vi "Test U8 Change FIFO Size.vi"() -> ()   [LabVIEW 2021]
uses:
  <vilib>/CIF Foundation/CIF Channels Core/ChannelCommon/typedef/Direction.ctl
  <vilib>/CIF Foundation/CIF Channels Core/ChannelCommon/typedef/TimeStamps.ctl
  CIF_CIPC_Fifo_U8.lvclass
  D:/dev/Packages/CIF_Channels_CIPC/src/CIPC_Channels/CIF_CIPC_Chan/CIF_CIPC_Chn.lvclass
  <vilib>/CIF Foundation/CIF Channels Core/ChannelCommon/typedef/New FIFO Instance Configuration.ctl
  <vilib>/CIF Foundation/CIF Channels Core/ChannelCommon/typedef/New FIFO Config.ctl
  <vilib>/CIF Foundation/CIF Channels Core/ChannelCommon/typedef/FIFO Flags.ctl
  <vilib>/CIF Foundation/CIF Channels Core/ChannelCommon/typedef/FIFO Config.ctl
  CIF_CIPC_Chan/CIF_CIPC_Chn.lvclass
  <vilib>/CIF Foundation/CIF Channels Core/ChannelCommon/ChannelCommon.lvlib
panel:
  out "status":string
  out "pass":bool
  out "error out":errorcluster
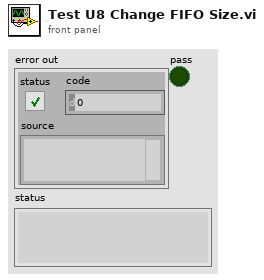
[diagram p1: front panel]
types:
  T1 = typedef "ChannelCommon.lvlib/Direction.ctl" = enum8{"Publisher", "Subscriber"}
  T2 = typedef "ChannelCommon.lvlib/New FIFO Config.ctl" = cluster{"Max Bytes/Msg":u64, "Max Msg/FIFO":u64, "FIFO Flags":T3, "Best Effort Subscribers":u32, "Backpressure Subscribers":u32}
  T3 = typedef "ChannelCommon.lvlib/FIFO Flags.ctl" = cluster{"Backpressure":bool, "Extended Config":bool}
  T4 = typedef "ChannelCommon.lvlib/New FIFO Instance Configuration.ctl" = cluster{"Backpressure":bool, "Bytes/Message Override":u32, "Messages/FIFO Override":u32, "Custom Data":u8[]}
  T5 = typedef "ChannelCommon.lvlib/TimeStamps.ctl" = cluster{"ClockID":u8, "T0":i64, "T_Out":i64}
  T6 = typedef "ChannelCommon.lvlib/FIFO Config.ctl" = cluster{"Max Bytes/Msg":u64, "Max Msg/FIFO":u64, "Flags":u64, "Custom Data":u8[]}
  T7 = typedef "ChannelCommon.lvlib/New FIFO Instance Response.ctl" = cluster{"Publisher":string, "Custom Data":u8[]}
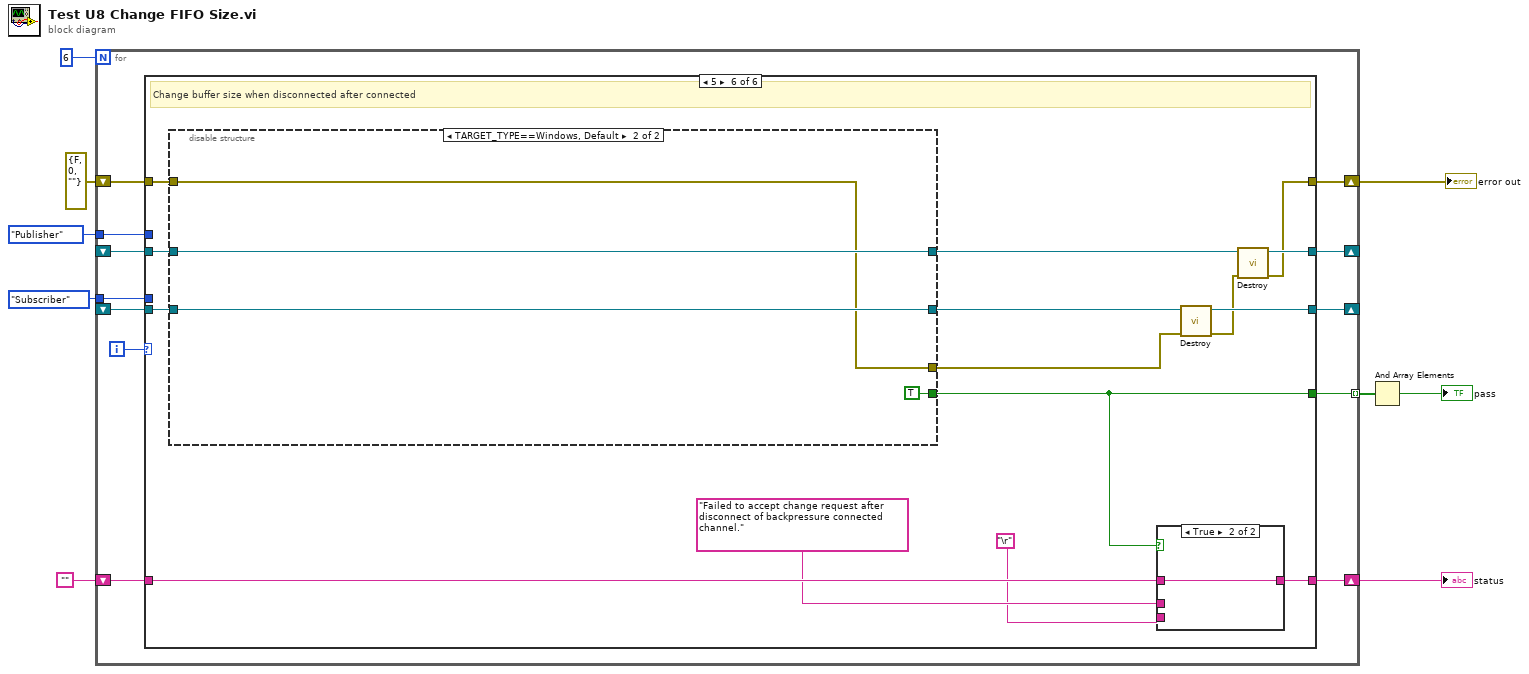
[diagram p0: block diagram]
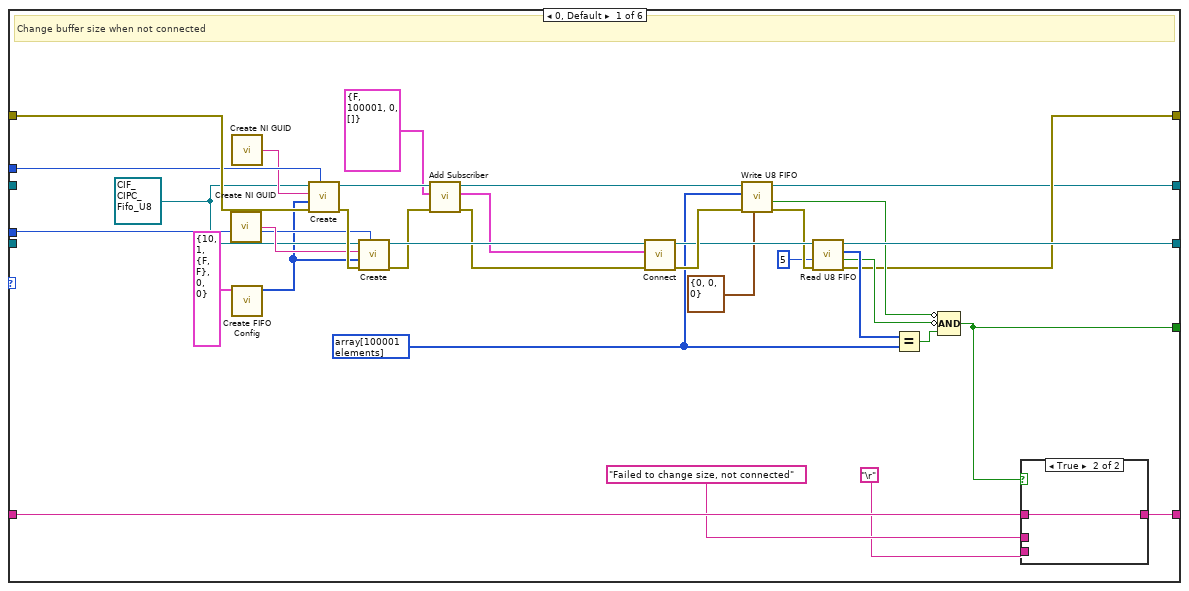
[diagram p2: hidden frame]
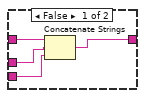
[diagram p3: hidden frame]
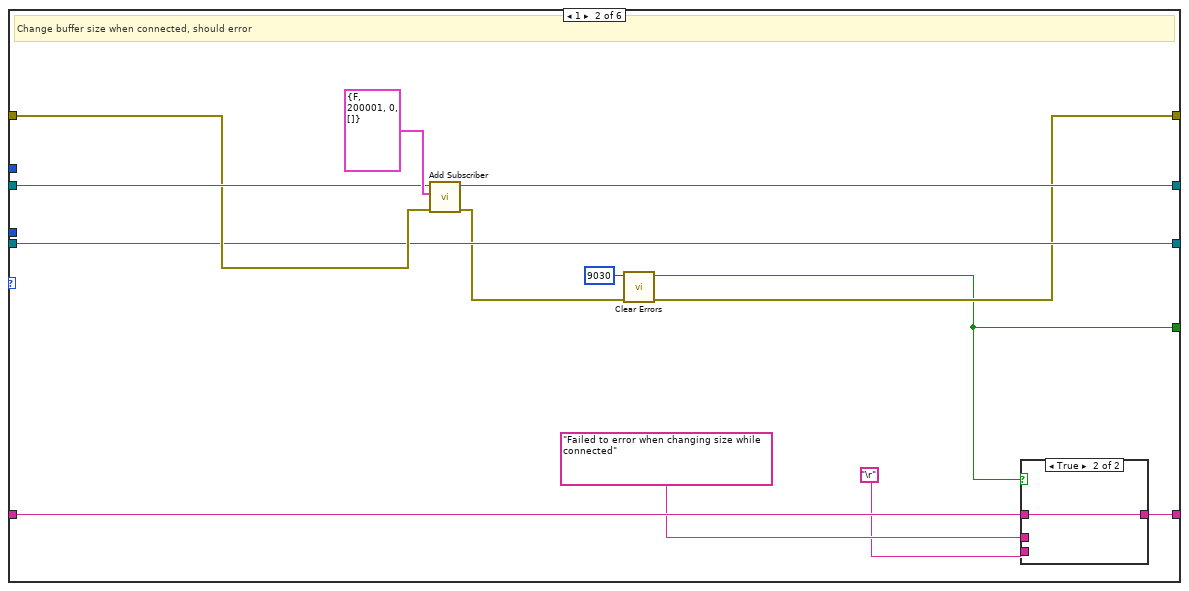
[diagram p4: hidden frame]
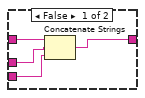
[diagram p5: hidden frame]
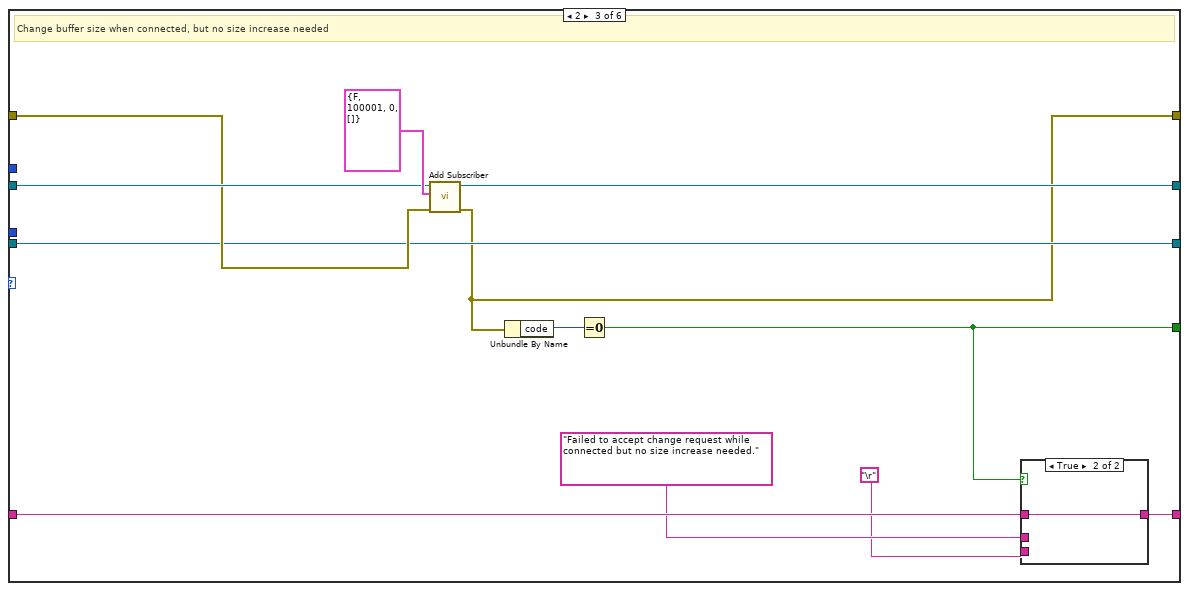
[diagram p6: hidden frame]
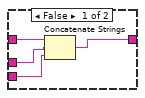
[diagram p7: hidden frame]
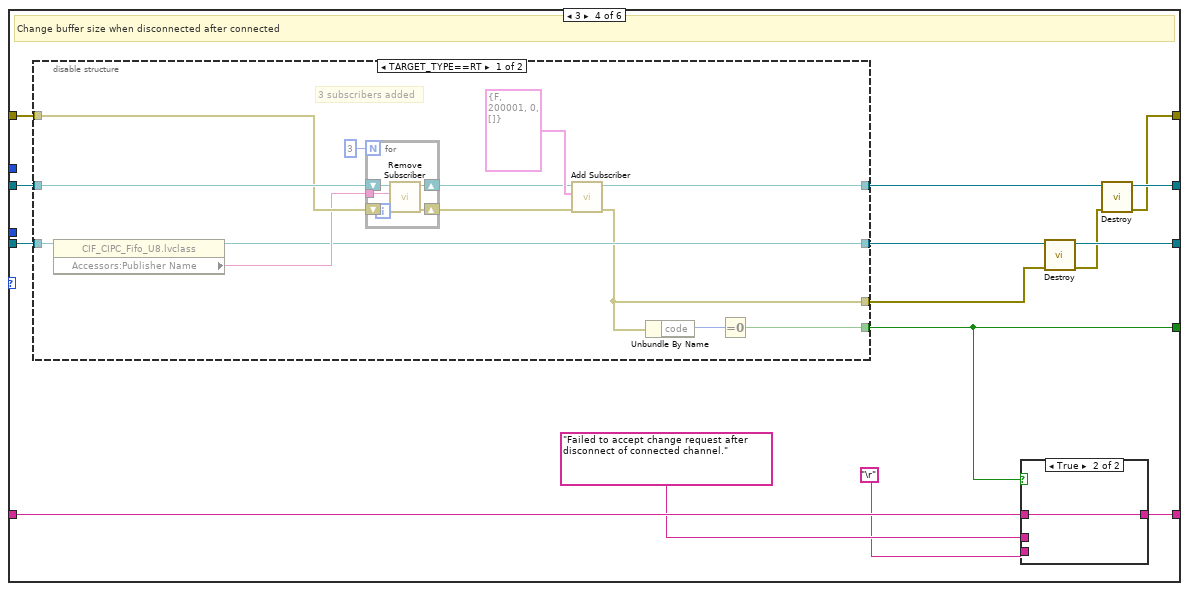
[diagram p8: hidden frame]
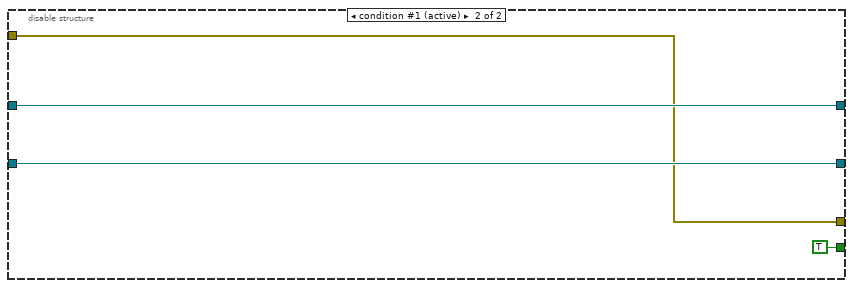
[diagram p9: hidden frame]
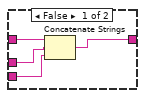
[diagram p10: hidden frame]
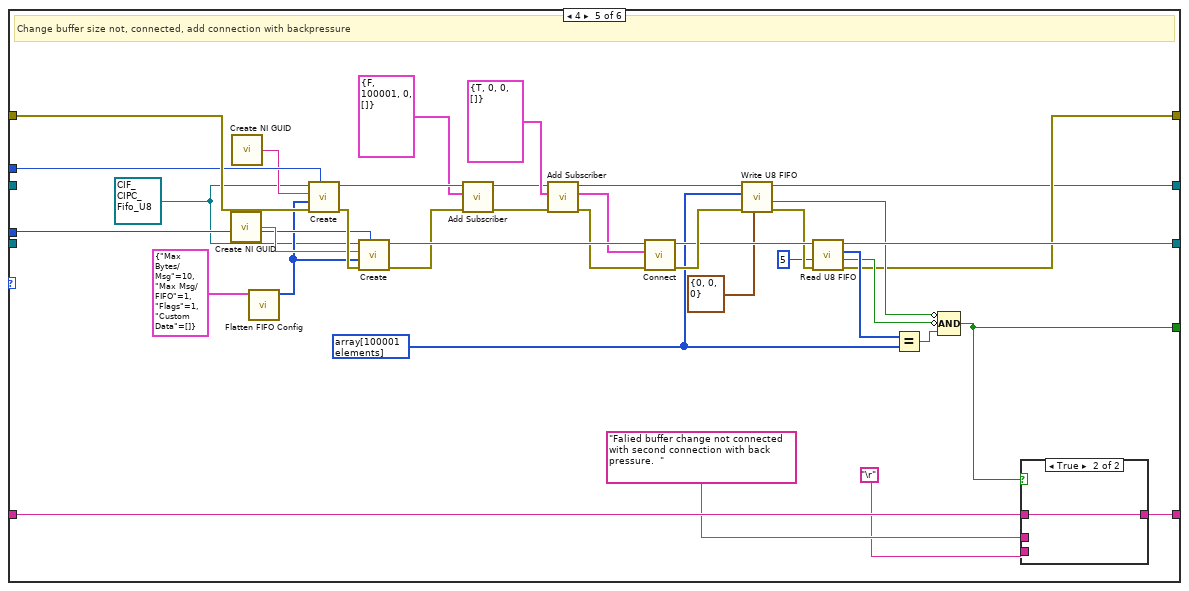
[diagram p11: hidden frame]
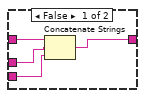
[diagram p12: hidden frame]
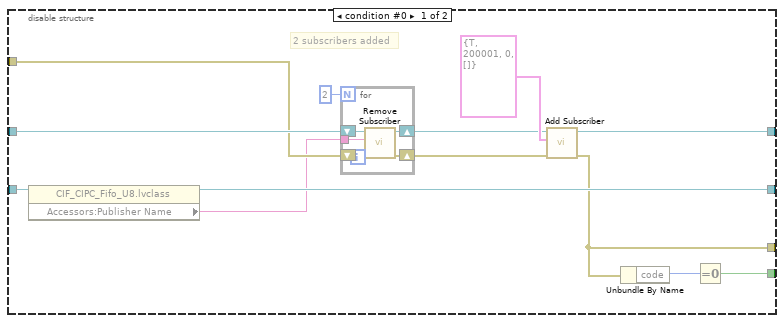
[diagram p13: hidden frame]
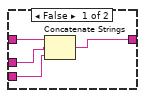
[diagram p14: hidden frame]
diagram:
  n1 = for {
    N: 6 -> [_]
    tunnel: [w21] -> w9 mode=indexing
    shift-right: [w19] -> w1
    shift-left: errorcluster {"status"=FALSE, "code"=0, "source"=""} ("error out") -> [w20]
    shift-right: [w16] -> w5
    shift-left: "" -> [w17]
    tunnel: Direction."Subscriber" ("Direction") -> [w15]
    tunnel: Direction."Publisher" ("Direction") -> [w14]
    shift-right: [w13] -> _
    shift-left: _ -> [w11]
    shift-right: [w12] -> _
    shift-left: _ -> [w10]
    i -> [w18]
    n2 = case shown="5" w18 {
      tunnel: [w50 w61 w79 w106 w169 w190] -> w21
      tunnel: w20 -> [w48 w67 w84 w104 w167 w188]
      tunnel: [w31 w63 w81 w96 w148 w180] -> w19
      tunnel: w17 -> [w55 w73 w90 w110 w174 w194]
      tunnel: [w54 w72 w89 w109 w173 w193] -> w16
      tunnel: w15 -> [w46 _ _ _ w165 _]
      tunnel: w14 -> [w45 _ _ _ w164 _]
      tunnel: [w40 w66 w83 w100 w158 w184] -> w13
      tunnel: [w30 w65 w82 w99 w147 w183] -> w12
      tunnel: w10 -> [_ w68 w85 w105 _ w189]
      tunnel: w11 -> [_ w66 w83 w103 _ w187]
      frame 0, Default {
        w35 = refnum<class "CIF_CIPC_Fifo_U8.lvclass"> refnum ("CIF_CIPC_Fifo_U8.lvclass")
        w32 = u8[] array[100001 elements] ("U8 Data")
        # "Change buffer size when not connected"
        n3 = call <vilib>:"Create NI GUID.vi"() -> ("NI GUID"=w47:string)
        n4 = call <vilib>:"Create NI GUID.vi"() -> ("NI GUID"=w44:string)
        n5 = call <vilib>:"Create FIFO Config.vi"("New FIFO Config"=T2 {"Max Bytes/Msg"=10, "Max Msg/FIFO"=1, "FIFO Flags"={"Backpressure"=FALSE, "Extended Config"=FALSE}, "Best Effort Subscribers"=0, "Backpressure Subscribers"=0}) -> ("Flattened FIFO Config"=w22:u8[])  [unwired: 10 in]
        n6 = call-dynamic "Create.vi"("Direction"=w45, "error in (no error)"=w48, "Custom Config Data"=w22, "Name"=w44, "CIFFIFO in"=w35) -> ("error out"=w49:errorcluster, "CIFFIFO out"=w29:refnum<class "CIF_CIPC_Fifo_U8.lvclass">)  [unwired: 5 in]
        n7 = call-dynamic "Create.vi"("Direction"=w46, "error in (no error)"=w49, "Custom Config Data"=w22, "Name"=w47, "CIFFIFO in"=w35) -> ("error out"=w25:errorcluster, "CIFFIFO out"=w43:refnum<class "CIF_CIPC_Fifo_U8.lvclass">)  [unwired: 5 in]
        n8 = call-dynamic "Add Subscriber.vi"("error in (no error)"=w25, "New FIFO Instance Config"=T4 {"Backpressure"=FALSE, "Bytes/Message Override"=100001, "Messages/FIFO Override"=0, "Custom Data"=[]}, "CIF_CIPC_Chn in"=w29) -> ("error out"=w24:errorcluster, "New FIFO Instance"=w27:T7, "CIF_CIPC_Chn out"=w28:refnum<class "CIF_CIPC_Fifo_U8.lvclass">)  [unwired: 6 in]
        n9 = call-dynamic "Connect.vi"("error in (no error)"=w24, "Connection"=w27, "CIFTag in"=w43) -> ("error out"=w42:errorcluster, "CIFTag out"=w41:refnum<class "CIF_CIPC_Fifo_U8.lvclass">)  [unwired: 7 in]
        n10 = call-dynamic "Write U8 FIFO.vi"("FIFO Timestamps"=T5 {"ClockID"=0, "T0"=0, "T_Out"=0}, "error in (no error)"=w42, "Data in"=w32, "CIFFIFO in"=w28) -> ("error out"=w39:errorcluster, "timed out?"=w38:bool, "CIFFIFO out"=w30:refnum<class "CIF_CIPC_Fifo_U8.lvclass">)  [unwired: 4 in, 1 out]
        n11 = call-dynamic "Read U8 FIFO.vi"("error in (no error)"=w39, "Timeout (ms)"=5, "CIFFIFO in"=w41) -> ("error out"=w31:errorcluster, "timed out?"=w36:bool, "Data out"=w37:u8[], "CIFFIFO out"=w40:refnum<class "CIF_CIPC_Fifo_U8.lvclass">)  [unwired: 4 in, 1 out]
        n12 = Equal?(x=w37, y=w32) -> (x = y?=w51:bool)
        n13 = Compound Arithmetic op=AND(invert w38, invert w36, w51) -> (w50:bool)
        n14 = case shown="True" w50 {
          tunnel: w55 -> [w59 w60]
          tunnel: [w56 w60] -> w54
          tunnel: "Failed to change size, not connected" -> [w58 _]
          tunnel: "\r" -> [w57 _]
          frame False {
            n15 = Concatenate Strings(w59, w58, w57) -> (w56:string)
          }
          frame True {
          }
        }
      }
      frame 1 {
        # "Change buffer size when connected, should error"
        n16 = call-dynamic "Add Subscriber.vi"("error in (no error)"=w67, "New FIFO Instance Config"=T4 {"Backpressure"=FALSE, "Bytes/Message Override"=200001, "Messages/FIFO Override"=0, "Custom Data"=[]}, "CIF_CIPC_Chn in"=w68) -> ("error out"=w64:errorcluster, "CIF_CIPC_Chn out"=w65:refnum<class "CIF_CIPC_Chn.lvclass">)  [unwired: 6 in, 1 out]
        n17 = call <vilib>:"Clear Errors.vi"("error in (no error)"=w64, "specific error code to clear (0: all)"=9030) -> ("error out"=w63:errorcluster, "specific error cleared?"=w61:bool)  [unwired: 4 in]
        n18 = case shown="True" w61 {
          tunnel: w73 -> [w77 w78]
          tunnel: [w74 w78] -> w72
          tunnel: "Failed to error when changing size while connected" -> [w76 _]
          tunnel: "\r" -> [w75 _]
          frame False {
            n19 = Concatenate Strings(w77, w76, w75) -> (w74:string)
          }
          frame True {
          }
        }
      }
      frame 2 {
        # "Change buffer size when connected, but no size increase needed"
        n20 = call-dynamic "Add Subscriber.vi"("error in (no error)"=w84, "New FIFO Instance Config"=T4 {"Backpressure"=FALSE, "Bytes/Message Override"=100001, "Messages/FIFO Override"=0, "Custom Data"=[]}, "CIF_CIPC_Chn in"=w85) -> ("error out"=w81:errorcluster, "CIF_CIPC_Chn out"=w82:refnum<class "CIF_CIPC_Chn.lvclass">)  [unwired: 6 in, 1 out]
        n21 = Unbundle By Name(w81) -> ("code"=w80:i32)
        n22 = Equal To 0?(x=w80) -> (x = 0?=w79:bool)
        n23 = case shown="True" w79 {
          tunnel: w90 -> [w94 w95]
          tunnel: [w91 w95] -> w89
          tunnel: "Failed to accept change request while connected but no size increase needed." -> [w93 _]
          tunnel: "\r" -> [w92 _]
          frame False {
            n24 = Concatenate Strings(w94, w93, w92) -> (w91:string)
          }
          frame True {
          }
        }
      }
      frame 3 {
        # "Change buffer size when disconnected after connected"
        n25 = disable-structure shown="TARGET_TYPE==RT" {
          disable-tunnel: [w121 TRUE] -> w106
          disable-tunnel: w105 -> [w120 w132]
          disable-tunnel: w104 -> [w117 w130]
          disable-tunnel: w103 -> [w116 w131]
          disable-tunnel: [w113 w132] -> w102
          disable-tunnel: [w112 w131] -> w101
          disable-tunnel: [w111 w130] -> w98
          frame condition #0 {
            # "3 subscribers added"
            n26 = property class="CIF_CIPC_Fifo_U8.lvclass"(reference=w116) -> (reference out=w112:refnum<class "CIF_CIPC_Fifo_U8.lvclass">, "Accessors:Publisher Name"=w115:string)  [unwired: 1 in, 1 out]
            n27 = for {
              N: 3 -> [_]
              tunnel: w115 -> [w124]
              shift-right: [w126] -> w118
              shift-left: w117 -> [w125]
              shift-right: [w127] -> w119
              shift-left: w120 -> [w128]
              n28 = call-dynamic "Remove Subscriber.vi"("error in (no error)"=w125, "Publisher to Remove"=w124, "CIF_CIPC_Chn in"=w128) -> ("error out"=w126:errorcluster, "CIF_CIPC_Chn out"=w127:refnum<class "CIF_CIPC_Chn.lvclass">)  [unwired: 7 in]
            }
            n29 = call-dynamic "Add Subscriber.vi"("error in (no error)"=w118, "New FIFO Instance Config"=T4 {"Backpressure"=FALSE, "Bytes/Message Override"=200001, "Messages/FIFO Override"=0, "Custom Data"=[]}, "CIF_CIPC_Chn in"=w119) -> ("error out"=w111:errorcluster, "CIF_CIPC_Chn out"=w113:refnum<class "CIF_CIPC_Chn.lvclass">)  [unwired: 6 in, 1 out]
            n30 = Unbundle By Name(w111) -> ("code"=w122:i32)
            n31 = Equal To 0?(x=w122) -> (x = 0?=w121:bool)
          }
          frame condition #1 (active) {
          }
        }
        n32 = case shown="True" w106 {
          tunnel: w110 -> [w136 w137]
          tunnel: [w133 w137] -> w109
          tunnel: "Failed to accept change request after disconnect of connected channel." -> [w135 _]
          tunnel: "\r" -> [w134 _]
          frame False {
            n33 = Concatenate Strings(w136, w135, w134) -> (w133:string)
          }
          frame True {
          }
        }
        n34 = call-dynamic "Destroy.vi"("error in (no error)"=w98, "CIFTag in"=w101) -> ("error out"=w97:errorcluster, "CIFTag out"=w100:refnum<class "CIF_CIPC_Fifo_U8.lvclass">)  [unwired: 8 in]
        n35 = call-dynamic "Destroy.vi"("error in (no error)"=w97, "CIFTag in"=w102) -> ("error out"=w96:errorcluster, "CIFTag out"=w99:refnum<class "CIF_CIPC_Chn.lvclass">)  [unwired: 8 in]
      }
      frame 4 {
        w152 = refnum<class "CIF_CIPC_Fifo_U8.lvclass"> refnum ("CIF_CIPC_Fifo_U8.lvclass")
        w149 = u8[] array[100001 elements] ("U8 Data")
        # "Change buffer size not, connected, add connection with backpressure"
        n36 = call <vilib>:"Create NI GUID.vi"() -> ("NI GUID"=w166:string)
        n37 = call <vilib>:"Create NI GUID.vi"() -> ("NI GUID"=w162:string)
        n38 = call <vilib>:"Flatten FIFO Config.vi"("FIFO Config in"=T6 {"Max Bytes/Msg"=10, "Max Msg/FIFO"=1, "Flags"=1, "Custom Data"=[]}) -> ("Flattened FIFO Config"=w153:u8[])  [unwired: 10 in]
        n39 = call-dynamic "Create.vi"("Direction"=w164, "error in (no error)"=w167, "Custom Config Data"=w153, "Name"=w162, "CIFFIFO in"=w152) -> ("error out"=w168:errorcluster, "CIFFIFO out"=w142:refnum<class "CIF_CIPC_Fifo_U8.lvclass">)  [unwired: 5 in]
        n40 = call-dynamic "Create.vi"("Direction"=w165, "error in (no error)"=w168, "Custom Config Data"=w153, "Name"=w166, "CIFFIFO in"=w152) -> ("error out"=w139:errorcluster, "CIFFIFO out"=w161:refnum<class "CIF_CIPC_Fifo_U8.lvclass">)  [unwired: 5 in]
        n41 = call-dynamic "Add Subscriber.vi"("error in (no error)"=w139, "New FIFO Instance Config"=T4 {"Backpressure"=FALSE, "Bytes/Message Override"=100001, "Messages/FIFO Override"=0, "Custom Data"=[]}, "CIF_CIPC_Chn in"=w142) -> ("error out"=w140:errorcluster, "CIF_CIPC_Chn out"=w141:refnum<class "CIF_CIPC_Fifo_U8.lvclass">)  [unwired: 6 in, 1 out]
        n42 = call-dynamic "Add Subscriber.vi"("error in (no error)"=w140, "New FIFO Instance Config"=T4 {"Backpressure"=TRUE, "Bytes/Message Override"=0, "Messages/FIFO Override"=0, "Custom Data"=[]}, "CIF_CIPC_Chn in"=w141) -> ("error out"=w143:errorcluster, "New FIFO Instance"=w145:T7, "CIF_CIPC_Chn out"=w146:refnum<class "CIF_CIPC_Fifo_U8.lvclass">)  [unwired: 6 in]
        n43 = call-dynamic "Connect.vi"("error in (no error)"=w143, "Connection"=w145, "CIFTag in"=w161) -> ("error out"=w160:errorcluster, "CIFTag out"=w159:refnum<class "CIF_CIPC_Fifo_U8.lvclass">)  [unwired: 7 in]
        n44 = call-dynamic "Write U8 FIFO.vi"("FIFO Timestamps"=T5 {"ClockID"=0, "T0"=0, "T_Out"=0}, "error in (no error)"=w160, "Data in"=w149, "CIFFIFO in"=w146) -> ("error out"=w157:errorcluster, "timed out?"=w156:bool, "CIFFIFO out"=w147:refnum<class "CIF_CIPC_Fifo_U8.lvclass">)  [unwired: 4 in, 1 out]
        n45 = call-dynamic "Read U8 FIFO.vi"("error in (no error)"=w157, "Timeout (ms)"=5, "CIFFIFO in"=w159) -> ("error out"=w148:errorcluster, "timed out?"=w154:bool, "Data out"=w155:u8[], "CIFFIFO out"=w158:refnum<class "CIF_CIPC_Fifo_U8.lvclass">)  [unwired: 4 in, 1 out]
        n46 = Equal?(x=w155, y=w149) -> (x = y?=w170:bool)
        n47 = Compound Arithmetic op=AND(invert w156, invert w154, w170) -> (w169:bool)
        n48 = case shown="True" w169 {
          tunnel: w174 -> [w178 w179]
          tunnel: [w175 w179] -> w173
          tunnel: "Falied buffer change not connected with second connection with back pressure.  " -> [w177 _]
          tunnel: "\r" -> [w176 _]
          frame False {
            n49 = Concatenate Strings(w178, w177, w176) -> (w175:string)
          }
          frame True {
          }
        }
      }
      frame 5 {
        # "Change buffer size when disconnected after connected"
        n50 = disable-structure shown="TARGET_TYPE==Windows, Default" {
          disable-tunnel: [w205 TRUE] -> w190
          disable-tunnel: w189 -> [w204 w216]
          disable-tunnel: w188 -> [w201 w214]
          disable-tunnel: w187 -> [w200 w215]
          disable-tunnel: [w198 w216] -> w186
          disable-tunnel: [w197 w215] -> w185
          disable-tunnel: [w196 w214] -> w182
          frame condition #0 {
            # "2 subscribers added"
            n51 = property class="CIF_CIPC_Fifo_U8.lvclass"(reference=w200) -> (reference out=w197:refnum<class "CIF_CIPC_Fifo_U8.lvclass">, "Accessors:Publisher Name"=w195:string)  [unwired: 1 in, 1 out]
            n52 = for {
              N: 2 -> [_]
              tunnel: w195 -> [w208]
              shift-right: [w210] -> w202
              shift-left: w201 -> [w209]
              shift-right: [w211] -> w203
              shift-left: w204 -> [w212]
              n53 = call-dynamic "Remove Subscriber.vi"("error in (no error)"=w209, "Publisher to Remove"=w208, "CIF_CIPC_Chn in"=w212) -> ("error out"=w210:errorcluster, "CIF_CIPC_Chn out"=w211:refnum<class "CIF_CIPC_Chn.lvclass">)  [unwired: 7 in]
            }
            n54 = call-dynamic "Add Subscriber.vi"("error in (no error)"=w202, "New FIFO Instance Config"=T4 {"Backpressure"=TRUE, "Bytes/Message Override"=200001, "Messages/FIFO Override"=0, "Custom Data"=[]}, "CIF_CIPC_Chn in"=w203) -> ("error out"=w196:errorcluster, "CIF_CIPC_Chn out"=w198:refnum<class "CIF_CIPC_Chn.lvclass">)  [unwired: 6 in, 1 out]
            n55 = Unbundle By Name(w196) -> ("code"=w206:i32)
            n56 = Equal To 0?(x=w206) -> (x = 0?=w205:bool)
          }
          frame condition #1 (active) {
          }
        }
        n57 = case shown="True" w190 {
          tunnel: w194 -> [w220 w221]
          tunnel: [w217 w221] -> w193
          tunnel: "Failed to accept change request after disconnect of backpressure connected channel." -> [w219 _]
          tunnel: "\r" -> [w218 _]
          frame False {
            n58 = Concatenate Strings(w220, w219, w218) -> (w217:string)
          }
          frame True {
          }
        }
        n59 = call-dynamic "Destroy.vi"("error in (no error)"=w182, "CIFTag in"=w185) -> ("error out"=w181:errorcluster, "CIFTag out"=w184:refnum<class "CIF_CIPC_Fifo_U8.lvclass">)  [unwired: 8 in]
        n60 = call-dynamic "Destroy.vi"("error in (no error)"=w181, "CIFTag in"=w186) -> ("error out"=w180:errorcluster, "CIFTag out"=w183:refnum<class "CIF_CIPC_Chn.lvclass">)  [unwired: 8 in]
      }
    }
  }
  "error out" <- w1
  "status" <- w5
  n61 = And Array Elements(Boolean array=w9) -> (logical AND=→"pass":bool)
